vi "2636 EPSC Pulse Sweep.vi"() -> ()   [LabVIEW 2023]
uses:
  <instrlib>/Keithley 2600 Series/Public/Channel.ctl
  <instrlib>/Keithley 2600 Series/Keithley 2600 Series.lvlib
  <userlib>/_OpenG.lib/time/time.llb/openg_time.lvlib
panel:
  in  "Pulse Level Step (V)":dbl=1.0
  in  "error in (no error)":errorcluster
  in  "Log Time After Pulses (s)":dbl=0.5 format="%#_13g"
  in  "Log Time Before Pulses (s)":dbl=0.5 format="%#_13g"
  in  "Auto Enable Output":bool=TRUE
  in  "Reset":bool=TRUE
  in  "Error Query":bool
  out "Pulsed IV Filename Out":path caption="Filename Out"
  in  "Pulsed IV Filename":path=path "C:/Data/pulse_I_V.lvm" caption="Filename"
  out "Pulse IV":cluster{"X":dbl[], "Y":dbl[]}[](graph)
  out "I_ds Log Filename Out":path caption="Filename Out"
  in  "I_ds Log Filename":path=path "C:/Data/I_ds_vs_time.lvm" caption="Filename"
  out "Data":dbl[](array[numeric])
  out "Result Chart":dynamicdata(graph)
  out "error out":errorcluster
  out "Complete?":bool
  out "Overflow?":bool
  in  "Stop":bool
  in  "Pulse Duration (s)":dbl=0.01
  in  "Post-Pulse Duration (s)":dbl=0.05
  in  "Pre-Pulse Duration (s)":dbl=0.05
  in  "Buffer size":u32=1024
  in  "Pulse Number":u32=10
  in  "Drain Source Channel":T1=enum."Channel B"
  in  "V_ds(V)":dbl=0.01
  in  "I_ds NPLC":dbl=0.1
  in  "I_ds Range (A)":dbl=1e-06
  in  "I pulse Range (A)":dbl=1e-06
  in  "I pulse NPLC":dbl=0.1
  in  "Pulse Level Start (V)":dbl=1.0
  in  "Pulse Channel":T1
  in  "2636 Address":refnum<visa-resource-name>="GPIB0::26::INSTR"
  # "Synaptic EPSC Pulse Sweep Measurement (Three-terminal Devices)"
  # "by JHC (20250322)"
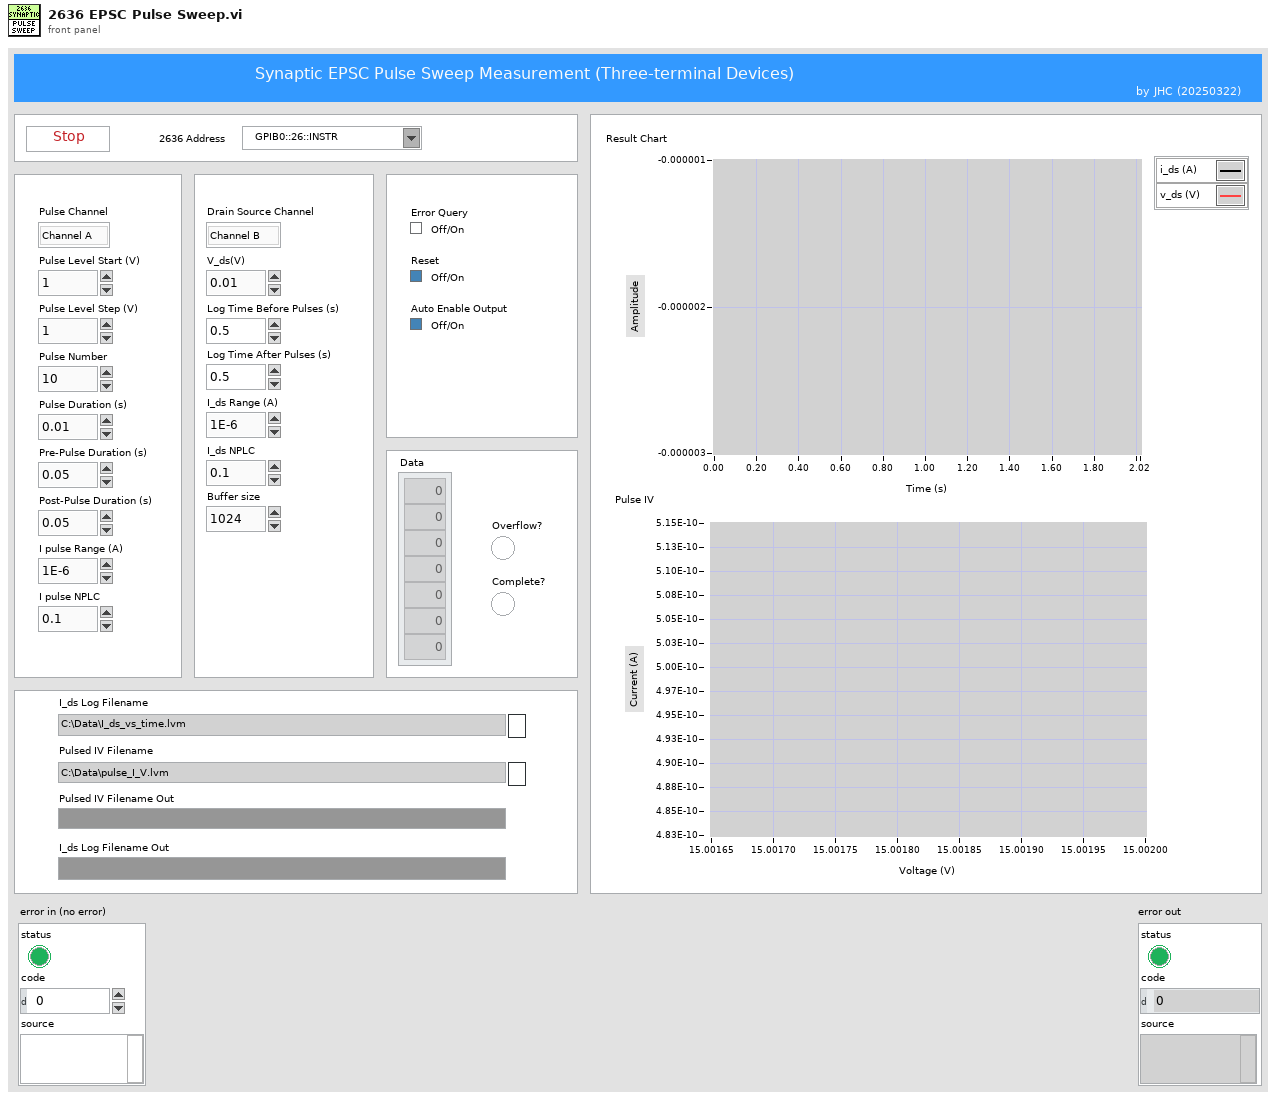
[diagram p1: front panel]
types:
  T1 = typedef "Keithley 2600 Series.lvlib/Channel.ctl" = enum32{"Channel A", "Channel B"}
  T2 = enum16{"None/Disconnect", "Digital I/O Trigger", "TSP-Link Trigger", "LAN Trigger", "Blender", "Timer Expired", "Front Panel Trigger", "Software Trigger", "SMU Sweeping", "SMU Armed", "SMU Source Complete", "SMU Measure Complete", "SMU Pulse Complete", "SMU Sweep Complete", "SMU Idle"}
  T3 = enum16{"Current", "Voltage", "IV", "Resistance", "Power"}
  T4 = enum32{"ASCII", "Real 32", "Real 64", "Single Precision Real", "Double Precision Real"}
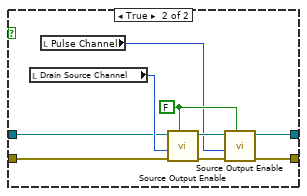
[diagram p2: hidden frame]
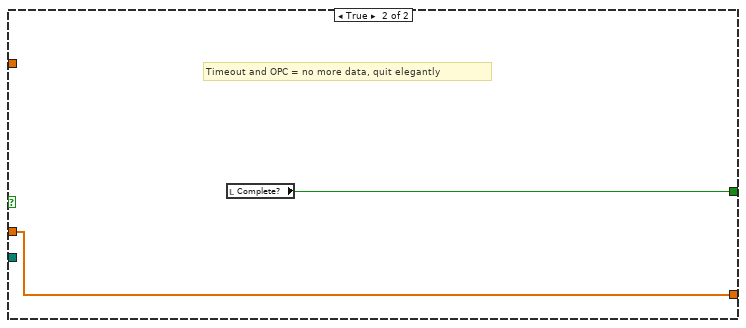
[diagram p5: hidden frame]
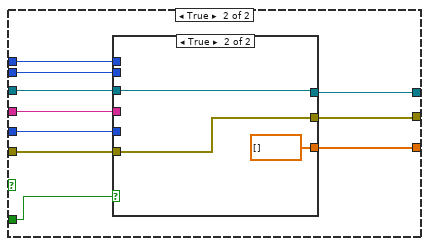
[diagram p8: hidden frame]
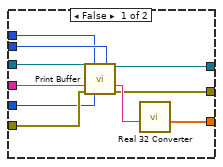
[diagram p9: hidden frame]
diagram:
  w19 = sgl[] [] ("Data Array Out")
  w22 = u16 1 items=["Channel A", "Channel B"] ("Channel (Channel A)")
  w23 = u16 0 items=["Channel A", "Channel B"] ("Channel (Channel A)")
  w39 = u16 0 items=["Current", "Voltage", "Resistance", "Power"] ("Function (Current)")
  w47 = u16 2 items=["Channel A", "Channel B", "Channels A & B", "User"] ("Screen (Channels A & B)")
  # "Wait 1s"
  # "Start Pulse SMU"
  # "Start DS SMU"
  n1 = call <instrlib>:"Initialize.vi"("Reset (True)"="Reset", "error in (no error)"="error in (no error)", "Error Query (False)"="Error Query", "ID Query (True)"=TRUE, "VISA resource name"="2636 Address") -> ("error out"=w2:errorcluster, "VISA resource name out"=w5:refnum<visa-resource-name>)  [unwired: 5 in]
  n2 = call <instrlib>:"Error Queue Clear.vi"("error in (no error)"=w2, "VISA resource name"=w5) -> ("error out"=w3:errorcluster, "VISA resource name out"=w4:refnum<visa-resource-name>)  [unwired: 6 in, 2 out]
  n3 = call <instrlib>:"Abort SMU Op.vi"("error in"=w3, "Channel (Channel A)"=w23, "VISA resource name"=w4) -> ("error out"=w24:errorcluster, "VISA resource name out"=w25:refnum<visa-resource-name>)  [unwired: 5 in, 2 out]
  n4 = call <instrlib>:"Abort SMU Op.vi"("error in"=w24, "Channel (Channel A)"=w22, "VISA resource name"=w25) -> ("error out"=w20:errorcluster, "VISA resource name out"=w21:refnum<visa-resource-name>)  [unwired: 5 in, 2 out]
  n5 = call <instrlib>:"Reset SMU.vi"("SMU B (No)"="Reset", "SMU A (No)"="Reset", "error in (no error)"=w20, "VISA resource name"=w21) -> ("error out"=w86:errorcluster, "VISA resource name out"=w87:refnum<visa-resource-name>)  [unwired: 4 in, 2 out]
  n6 = flat-sequence {
    tunnel: w87 -> [w120]
    tunnel: w86 -> [w119]
    tunnel: [w101] -> w85
    tunnel: [w100] -> w84
    tunnel: w85 -> [w143]
    tunnel: w84 -> [w144]
    tunnel: [w142] -> w83
    tunnel: [w141] -> w82
    tunnel: w83 -> [w185]
    tunnel: w82 -> [w183]
    tunnel: [w164] -> w81
    tunnel: [w163] -> w80
    tunnel: w81 -> [w269]
    tunnel: w80 -> [w268]
    tunnel: [w236] -> w79
    tunnel: [w235] -> w78
    tunnel: [w221] -> w77
    tunnel: w79 -> [w306]
    tunnel: w78 -> [w307]
    tunnel: w77 -> [w329]
    tunnel: [w310] -> w76
    tunnel: [w309] -> w75
    tunnel: w76 -> [w337]
    tunnel: w75 -> [w336]
    tunnel: [w333] -> w44
    tunnel: [w332] -> w43
    frame #0 {
      w108 = enum32{"Current", "Voltage"}."Current" ("Function (Current)")
      w109 = FALSE ("Autorange (On)")
      w89 = enum32{"Current", "Voltage"}."Voltage" ("Function (Current)")
      # "Init Pulse Gate Channel"
      n7 = call <instrlib>:"Source Function.vi"("Function (Current)"=w89, "error in (no error)"=w119, "Channel (Channel A)"="Pulse Channel", "VISA resource name"=w120) -> ("error out"=w121:errorcluster, "VISA resource name out"=w122:refnum<visa-resource-name>)  [unwired: 4 in, 2 out]
      n8 = call <instrlib>:"Source Level.vi"("Level (0.000)"=0.0, "Function (Current)"=w89, "error in (no error)"=w121, "Channel (Channel A)"="Pulse Channel", "VISA resource name"=w122) -> ("error out"=w117:errorcluster, "VISA resource name out"=w118:refnum<visa-resource-name>)  [unwired: 3 in, 2 out]
      n9 = call <instrlib>:"Source Autorange.vi"("Autorange (On)"=w109, "Function (Current)"=w89, "error in (no error)"=w117, "Channel (Channel A)"="Pulse Channel", "VISA resource name"=w118) -> ("error out"=w115:errorcluster, "VISA resource name out"=w116:refnum<visa-resource-name>)  [unwired: 3 in, 2 out]
      n10 = local read "Pulse Level Start (V)"() -> (w88:dbl)
      n11 = call <instrlib>:"Source Autorange.vi"("Autorange (On)"=w109, "Function (Current)"=w108, "error in (no error)"=w115, "Channel (Channel A)"="Pulse Channel", "VISA resource name"=w116) -> ("error out"=w96:errorcluster, "VISA resource name out"=w98:refnum<visa-resource-name>)  [unwired: 3 in, 2 out]
      n12 = call <instrlib>:"Source Range.vi"("Range (1.000)"=w88, "Function (Current)"=w89, "error in (no error)"=w96, "Channel (Channel A)"="Pulse Channel", "VISA resource name"=w98) -> ("error out"=w95:errorcluster, "VISA resource name out"=w97:refnum<visa-resource-name>)  [unwired: 3 in, 2 out]
      n13 = call <instrlib>:"Measure NPLC.vi"("NPLC (1.000)"="I pulse NPLC", "error in (no error)"=w95, "Channel (Channel A)"="Pulse Channel", "VISA resource name"=w97) -> ("error out"=w113:errorcluster, "VISA resource name out"=w110:refnum<visa-resource-name>)  [unwired: 4 in, 2 out]
      n14 = call <instrlib>:"Measure Autorange.vi"("Autorange (On)"=w109, "Function (Current)"=w89, "error in (no error)"=w113, "Channel (Channel A)"="Pulse Channel", "VISA resource name"=w110) -> ("error out"=w112:errorcluster, "VISA resource name out"=w111:refnum<visa-resource-name>)  [unwired: 3 in, 2 out]
      n15 = call <instrlib>:"Measure Autorange.vi"("Autorange (On)"=w109, "Function (Current)"=w108, "error in (no error)"=w112, "Channel (Channel A)"="Pulse Channel", "VISA resource name"=w111) -> ("error out"=w94:errorcluster, "VISA resource name out"=w93:refnum<visa-resource-name>)  [unwired: 3 in, 2 out]
      n16 = call <instrlib>:"Measure Range.vi"("Range (1.000)"=w88, "Function (Current)"=w89, "error in (no error)"=w94, "Channel (Channel A)"="Pulse Channel", "VISA resource name"=w93) -> ("error out"=w91:errorcluster, "VISA resource name out"=w92:refnum<visa-resource-name>)  [unwired: 3 in, 2 out]
      n17 = call <instrlib>:"Measure Range.vi"("Range (1.000)"="I pulse Range (A)", "Function (Current)"=w108, "error in (no error)"=w91, "Channel (Channel A)"="Pulse Channel", "VISA resource name"=w92) -> ("error out"=w106:errorcluster, "VISA resource name out"=w105:refnum<visa-resource-name>)  [unwired: 3 in, 2 out]
      n18 = call <instrlib>:"Measure Sense Mode.vi"("error in (no error)"=w106, "Channel (Channel A)"="Pulse Channel", "VISA resource name"=w105) -> ("error out"=w103:errorcluster, "VISA resource name out"=w104:refnum<visa-resource-name>)  [unwired: 2 in, 5 out]
      n19 = call <instrlib>:"Measure Autozero.vi"("Autozero (Auto)"=enum32{"Off", "Once", "Auto"}."Once", "error in (no error)"=w103, "Channel (Channel A)"="Pulse Channel", "VISA resource name"=w104) -> ("error out"=w100:errorcluster, "VISA resource name out"=w101:refnum<visa-resource-name>)  [unwired: 1 in, 5 out]
    }
    frame #1 {
      w126 = 0.0 ("Interval (0.000)")
      w146 = enum32{"Current", "Voltage"}."Current" ("Function (Current)")
      w145 = FALSE ("Autorange (On)")
      w132 = enum32{"Current", "Voltage"}."Voltage" ("Function (Current)")
      # "Init Drain Source Channel"
      n20 = call <instrlib>:"Source Function.vi"("Function (Current)"=w132, "error in (no error)"=w144, "Channel (Channel A)"="Drain Source Channel", "VISA resource name"=w143) -> ("error out"=w160:errorcluster, "VISA resource name out"=w161:refnum<visa-resource-name>)  [unwired: 4 in, 2 out]
      n21 = call <instrlib>:"Source Level.vi"("Level (0.000)"="V_ds(V)", "Function (Current)"=w132, "error in (no error)"=w160, "Channel (Channel A)"="Drain Source Channel", "VISA resource name"=w161) -> ("error out"=w158:errorcluster, "VISA resource name out"=w159:refnum<visa-resource-name>)  [unwired: 3 in, 2 out]
      n22 = call <instrlib>:"Source Autorange.vi"("Autorange (On)"=w145, "Function (Current)"=w132, "error in (no error)"=w158, "Channel (Channel A)"="Drain Source Channel", "VISA resource name"=w159) -> ("error out"=w156:errorcluster, "VISA resource name out"=w157:refnum<visa-resource-name>)  [unwired: 3 in, 2 out]
      n23 = call <instrlib>:"Source Autorange.vi"("Autorange (On)"=w145, "Function (Current)"=w146, "error in (no error)"=w156, "Channel (Channel A)"="Drain Source Channel", "VISA resource name"=w157) -> ("error out"=w140:errorcluster, "VISA resource name out"=w137:refnum<visa-resource-name>)  [unwired: 3 in, 2 out]
      n24 = call <instrlib>:"Source Range.vi"("Range (1.000)"="V_ds(V)", "Function (Current)"=w132, "error in (no error)"=w140, "Channel (Channel A)"="Drain Source Channel", "VISA resource name"=w137) -> ("error out"=w139:errorcluster, "VISA resource name out"=w138:refnum<visa-resource-name>)  [unwired: 3 in, 2 out]
      n25 = call <instrlib>:"Measure NPLC.vi"("NPLC (1.000)"="I_ds NPLC", "error in (no error)"=w139, "Channel (Channel A)"="Drain Source Channel", "VISA resource name"=w138) -> ("error out"=w127:errorcluster, "VISA resource name out"=w128:refnum<visa-resource-name>)  [unwired: 4 in, 2 out]
      n26 = call <instrlib>:"Measure Interval.vi"("Interval (0.000)"=w126, "error in (no error)"=w127, "Channel (Channel A)"="Drain Source Channel", "VISA resource name"=w128) -> ("error out"=w130:errorcluster, "VISA resource name out"=w129:refnum<visa-resource-name>)  [unwired: 4 in, 2 out]
      n27 = call <instrlib>:"Measure Delay.vi"("Delay (0)"=w126, "error in (no error)"=w130, "Channel (Channel A)"="Drain Source Channel", "VISA resource name"=w129) -> ("error out"=w124:errorcluster, "VISA resource name out"=w125:refnum<visa-resource-name>)  [unwired: 4 in, 2 out]
      n28 = call <instrlib>:"Measure Autorange.vi"("Autorange (On)"=w145, "Function (Current)"=w132, "error in (no error)"=w124, "Channel (Channel A)"="Drain Source Channel", "VISA resource name"=w125) -> ("error out"=w154:errorcluster, "VISA resource name out"=w153:refnum<visa-resource-name>)  [unwired: 3 in, 2 out]
      n29 = call <instrlib>:"Measure Autorange.vi"("Autorange (On)"=w145, "Function (Current)"=w146, "error in (no error)"=w154, "Channel (Channel A)"="Drain Source Channel", "VISA resource name"=w153) -> ("error out"=w133:errorcluster, "VISA resource name out"=w134:refnum<visa-resource-name>)  [unwired: 3 in, 2 out]
      n30 = call <instrlib>:"Measure Range.vi"("Range (1.000)"="V_ds(V)", "Function (Current)"=w132, "error in (no error)"=w133, "Channel (Channel A)"="Drain Source Channel", "VISA resource name"=w134) -> ("error out"=w136:errorcluster, "VISA resource name out"=w135:refnum<visa-resource-name>)  [unwired: 3 in, 2 out]
      n31 = call <instrlib>:"Measure Range.vi"("Range (1.000)"="I_ds Range (A)", "Function (Current)"=w146, "error in (no error)"=w136, "VISA resource name"=w135) -> ("error out"=w151:errorcluster, "VISA resource name out"=w150:refnum<visa-resource-name>)  [unwired: 4 in, 2 out]
      n32 = call <instrlib>:"Measure Sense Mode.vi"("error in (no error)"=w151, "Channel (Channel A)"="Drain Source Channel", "VISA resource name"=w150) -> ("error out"=w148:errorcluster, "VISA resource name out"=w149:refnum<visa-resource-name>)  [unwired: 2 in, 5 out]
      n33 = call <instrlib>:"Measure Autozero.vi"("Autozero (Auto)"=enum32{"Off", "Once", "Auto"}."Once", "error in (no error)"=w148, "Channel (Channel A)"="Drain Source Channel", "VISA resource name"=w149) -> ("error out"=w142:errorcluster, "VISA resource name out"=w141:refnum<visa-resource-name>)  [unwired: 1 in, 5 out]
    }
    frame #2 {
      w177 = TRUE ("Append Mode (Off)")
      w176 = "v_ds" ("Buffer Name (buf)")
      w178 = TRUE ("Append Mode (Off)")
      w180 = "i_ds" ("Buffer Name (buf)")
      w189 = FALSE ("Collect Timestamps (Off)")
      w188 = "pulse_iv_table.v" ("Buffer Name (buf)")
      w187 = TRUE ("Append Mode (Off)")
      w186 = "pulse_iv_table.i" ("Buffer Name (buf)")
      # "set up circular buffer"
      # "A large size"
      # "Init Buffer"
      n34 = local read "Pulse Channel"() -> (w204:T1)
      n35 = VISA Write(VISA resource name=w183, write buffer="pulse_iv_table = {}\nds_iv_table = {}", error in (no error)=w185) -> (VISA resource name out=w190:refnum<visa-resource-name>, error out=w191:errorcluster)  [unwired: 1 out]
      n36 = local read "Pulse Number"() -> (w162:u32)
      n37 = call <instrlib>:"Error Query.vi"("error in (no error)"=w191, "VISA resource name"=w190) -> ("error out"=w203:errorcluster, "VISA resource name out"=w202:refnum<visa-resource-name>)  [unwired: 8 out]
      n38 = call <instrlib>:"Buffer Make Buffer.vi"("Capacity (1)"=w162, "Channel (Channel A)"=w204, "error in (no error)"=w203, "Buffer Name (buf)"=w186, "VISA resource name"=w202) -> ("error out"=w192:errorcluster, "VISA resource name out"=w193:refnum<visa-resource-name>)  [unwired: 1 in, 4 out]
      n39 = call <instrlib>:"Buffer Clear.vi"("error in (no error)"=w192, "Buffer Name"=w186, "VISA resource name"=w193) -> ("error out"=w195:errorcluster, "VISA resource name out"=w194:refnum<visa-resource-name>)  [unwired: 7 out]
      n40 = call <instrlib>:"Buffer Configure.vi"("Collect Timestamps (Off)"=w189, "error in (no error)"=w195, "Buffer Name"=w186, "Append Mode (Off)"=w187, "VISA resource name"=w194) -> ("error out"=w197:errorcluster, "VISA resource name out"=w196:refnum<visa-resource-name>)  [unwired: 2 in, 3 out]
      n41 = call <instrlib>:"Buffer Make Buffer.vi"("Capacity (1)"=w162, "Channel (Channel A)"=w204, "error in (no error)"=w197, "Buffer Name (buf)"=w188, "VISA resource name"=w196) -> ("error out"=w199:errorcluster, "VISA resource name out"=w198:refnum<visa-resource-name>)  [unwired: 1 in, 4 out]
      n42 = call <instrlib>:"Buffer Clear.vi"("error in (no error)"=w199, "Buffer Name"=w188, "VISA resource name"=w198) -> ("error out"=w201:errorcluster, "VISA resource name out"=w200:refnum<visa-resource-name>)  [unwired: 7 out]
      n43 = call <instrlib>:"Buffer Configure.vi"("Collect Source Values (Off)"=w189, "error in (no error)"=w201, "Buffer Name"=w188, "Append Mode (Off)"=w187, "VISA resource name"=w200) -> ("error out"=w210:errorcluster, "VISA resource name out"=w209:refnum<visa-resource-name>)  [unwired: 2 in, 3 out]
      n44 = local read "Drain Source Channel"() -> (w168:T1)
      n45 = call <instrlib>:"Buffer Make Buffer.vi"("Capacity (1)"="Buffer size", "Channel (Channel A)"=w168, "error in (no error)"=w210, "Buffer Name (buf)"=w180, "VISA resource name"=w209) -> ("error out"=w206:errorcluster, "VISA resource name out"=w205:refnum<visa-resource-name>)  [unwired: 1 in, 4 out]
      n46 = call <instrlib>:"Buffer Clear.vi"("error in (no error)"=w206, "Buffer Name"=w180, "VISA resource name"=w205) -> ("error out"=w208:errorcluster, "VISA resource name out"=w207:refnum<visa-resource-name>)  [unwired: 7 out]
      n47 = call <instrlib>:"Buffer Configure.vi"("Collect Timestamps (Off)"=w178, "error in (no error)"=w208, "Buffer Name"=w180, "Append Mode (Off)"=w178, "VISA resource name"=w207) -> ("error out"=w182:errorcluster, "VISA resource name out"=w181:refnum<visa-resource-name>)  [unwired: 2 in, 3 out]
      n48 = call <instrlib>:"Advanced Buffer Configuration.vi"("VISA resource name"=w181, "Enable Buffer Cache Mode (Disable)"=w178, "Buffer Name"=w180, "Buffer Fill Mode (Fill_Once)"=enum16{"FILL_ONCE", "FILL_WINDOW"}."FILL_WINDOW", "error in (no error)"=w182) -> ("VISA resource name out"=w166:refnum<visa-resource-name>, "error out"=w165:errorcluster)  [unwired: 9 in]
      n49 = call <instrlib>:"Buffer Make Buffer.vi"("Capacity (1)"="Buffer size", "Channel (Channel A)"=w168, "error in (no error)"=w165, "Buffer Name (buf)"=w176, "VISA resource name"=w166) -> ("error out"=w172:errorcluster, "VISA resource name out"=w173:refnum<visa-resource-name>)  [unwired: 1 in, 4 out]
      n50 = call <instrlib>:"Buffer Clear.vi"("error in (no error)"=w172, "Buffer Name"=w176, "VISA resource name"=w173) -> ("error out"=w170:errorcluster, "VISA resource name out"=w171:refnum<visa-resource-name>)  [unwired: 7 out]
      n51 = call <instrlib>:"Buffer Configure.vi"("Collect Timestamps (Off)"=w177, "error in (no error)"=w170, "Buffer Name"=w176, "Append Mode (Off)"=w177, "VISA resource name"=w171) -> ("error out"=w174:errorcluster, "VISA resource name out"=w175:refnum<visa-resource-name>)  [unwired: 2 in, 3 out]
      n52 = call <instrlib>:"Advanced Buffer Configuration.vi"("VISA resource name"=w175, "Enable Buffer Cache Mode (Disable)"=w177, "Buffer Name"=w176, "Buffer Fill Mode (Fill_Once)"=enum16{"FILL_ONCE", "FILL_WINDOW"}."FILL_WINDOW", "error in (no error)"=w174) -> ("VISA resource name out"=w163:refnum<visa-resource-name>, "error out"=w164:errorcluster)  [unwired: 9 in]
    }
    frame #3 {
      w225 = u32 4 ("Timer Number (1)")
      w239 = u32 1 ("Timer Number (1)")
      w251 = u32 3 ("Timer Number (1)")
      w274 = u32 2 ("Timer Number (1)")
      # "SMU Armed when timer4 expires"
      # "Trigger timer4 when the SMU Sweeping, only once"
      # "Trigger timer1 when the SMU Armed, repeat N times"
      # "Trigger end pulse after timer3 expired"
      # "Configure measure action (default is 0) to start after source immediately"
      # "set source pulse level and end pusle idle"
      # "Trigger timer3 when the SMU source pulse level"
      # "Create a fixed level voltage sweep"
      # "Configure source action to start after timer2 expired"
      # "Trigger timer2 when timer1 expired or first run."
      # "Init Trigger Model (Pulse Channel)"
      n53 = for {
        N: "Pulse Number" -> [_]
        tunnel: "Pulse Level Start (V)" -> [w284]
        tunnel: "Pulse Level Step (V)" -> [w285]
        tunnel: [w282] -> w212 mode=indexing
        i -> [w286]
        n54 = Multiply(x=w285, y=w286) -> (x*y=w283:dbl)
        n55 = Add(x=w284, y=w283) -> (x+y=w282:dbl)
      }
      n56 = Array To Spreadsheet String(delimiter (Tab)=",", array=w212, 3:"%f" ("format string")) -> (spreadsheet string=w211:string)
      n57 = local read "Pulse Channel"() -> (w221:T1)
      n58 = Pick Line(multi-line string="smua\nsmub", line index=w221) -> (output string=w234:string)  [unwired: 1 in]
      n59 = Format Into String(format string="%s.trigger.source.listv({%s})\\n", w234, w211) -> (resulting string=w272:string)  [unwired: 2 in, 1 out]
      n60 = call <instrlib>:"Format Event ID.vi"("Channel (Channel A)"=w221, "Event Type (None)"=T2."SMU Sweeping") -> ("Event ID"=w229:string)  [unwired: 8 in, 1 out]
      n61 = Format Into String(format string="%s.trigger.source.action = %s.ENABLE\n%s.trigger.endpulse.action = %s.SOURCE_IDLE", initial string=w272, w234, w234, w234, w234) -> (resulting string=w267:string)  [unwired: 1 in, 1 out]
      n62 = VISA Write(VISA resource name=w268, write buffer=w267, error in (no error)=w269) -> (VISA resource name out=w231:refnum<visa-resource-name>, error out=w230:errorcluster)  [unwired: 1 out]
      n63 = call <instrlib>:"Config Timer.vi"("VISA resource name"=w231, "Delay (1e-3)"="Log Time Before Pulses (s)", "Timer Number (1)"=w225, "error in"=w230, "Input Event"=w229) -> ("VISA resource name out"=w227:refnum<visa-resource-name>, "error out"=w223:errorcluster)  [unwired: 7 in, 2 out]
      n64 = call <instrlib>:"Format Event ID.vi"("Event Module # (1)"=w225, "Event Type (None)"=T2."Timer Expired") -> ("Event ID"=w224:string)  [unwired: 8 in, 1 out]
      n65 = call <instrlib>:"Config Arm Event.vi"("Arm Input Event"=w224, "error in"=w223, "Channel (Channel A)"=w221, "VISA resource name"=w227) -> ("error out"=w219:errorcluster, "VISA resource name out"=w218:refnum<visa-resource-name>)  [unwired: 4 in, 2 out]
      n66 = call <instrlib>:"Format Event ID.vi"("Channel (Channel A)"=w221, "Event Type (None)"=T2."SMU Armed") -> ("Event ID"=w220:string)  [unwired: 8 in, 1 out]
      n67 = local read "Pre-Pulse Duration (s)"() -> (w248:dbl)
      n68 = local read "Pulse Number"() -> (w244:u32)
      n69 = local read "Pulse Duration (s)"() -> (w249:dbl)
      n70 = Decrement(x=w244) -> (x-1=w240:u32)
      n71 = Compound Arithmetic op=ADD(w249, w248, "Post-Pulse Duration (s)") -> (w246:dbl)
      n72 = call <instrlib>:"Config Timer.vi"("VISA resource name"=w218, "Count (1)"=w240, "Delay (1e-3)"=w246, "Timer Number (1)"=w239, "Passthrough (Off)"=TRUE, "error in"=w219, "Input Event"=w220) -> ("VISA resource name out"=w241:refnum<visa-resource-name>, "error out"=w242:errorcluster)  [unwired: 5 in, 2 out]
      n73 = call <instrlib>:"Format Event ID.vi"("Event Module # (1)"=w239, "Event Type (None)"=T2."Timer Expired") -> ("Event ID"=w278:string)  [unwired: 8 in, 1 out]
      n74 = call <instrlib>:"Config Timer.vi"("VISA resource name"=w241, "Delay (1e-3)"="Pre-Pulse Duration (s)", "Timer Number (1)"=w274, "error in"=w242, "Input Event"=w278) -> ("VISA resource name out"=w277:refnum<visa-resource-name>, "error out"=w276:errorcluster)  [unwired: 7 in, 2 out]
      n75 = call <instrlib>:"Format Event ID.vi"("Event Module # (1)"=w274, "Event Type (None)"=T2."Timer Expired") -> ("Event ID"=w273:string)  [unwired: 8 in, 1 out]
      n76 = call <instrlib>:"Config Source Event.vi"("Input Event"=w273, "error in"=w276, "Channel (Channel A)"=w221, "VISA resource name"=w277) -> ("error out"=w262:errorcluster, "VISA resource name out"=w263:refnum<visa-resource-name>)  [unwired: 4 in, 2 out]
      n77 = call <instrlib>:"Format Event ID.vi"("Channel (Channel A)"=w221, "Event Type (None)"=T2."SMU Source Complete") -> ("Event ID"=w265:string)  [unwired: 8 in, 1 out]
      n78 = call <instrlib>:"Config Timer.vi"("VISA resource name"=w263, "Delay (1e-3)"="Pulse Duration (s)", "Timer Number (1)"=w251, "error in"=w262, "Input Event"=w265) -> ("VISA resource name out"=w261:refnum<visa-resource-name>, "error out"=w260:errorcluster)  [unwired: 7 in, 2 out]
      n79 = call <instrlib>:"Config Measure Event.vi"("VISA resource name"=w261, "Configure Measurement (Disable)"=enum8{"DISABLE", "ENABLE", "ASYNC"}."ENABLE", "Buffer 1"="pulse_iv_table.i" ("Buffer Name (buf)"), "Buffer 2"="pulse_iv_table.v" ("Buffer Name (buf)"), "Channel (Channel A)"=w221, "Function (Current)"=T3."IV", "error in"=w260, "Measure Input Event"="0") -> ("VISA resource name out"=w254:refnum<visa-resource-name>, "error out"=w253:errorcluster)  [unwired: 4 in, 2 out]
      n80 = call <instrlib>:"Format Event ID.vi"("Event Module # (1)"=w251, "Event Type (None)"=T2."Timer Expired") -> ("Event ID"=w250:string)  [unwired: 8 in, 1 out]
      n81 = local read "Pulse Number"() -> (w232:u32)
      n82 = call <instrlib>:"Config End Pulse Event.vi"("Input Event"=w250, "error in"=w253, "Channel (Channel A)"=w221, "VISA resource name"=w254) -> ("error out"=w238:errorcluster, "VISA resource name out"=w237:refnum<visa-resource-name>)  [unwired: 4 in, 2 out]
      n83 = call <instrlib>:"Config Layer Count.vi"("Trigger Count (1)"=w232, "Arm Count (1)"=u32 1 ("Trigger Count (1)"), "error in"=w238, "Channel (Channel A)"=w221, "VISA resource name"=w237) -> ("error out"=w235:errorcluster, "VISA resource name out"=w236:refnum<visa-resource-name>)  [unwired: 3 in, 2 out]
    }
    frame #4 {
      w291 = u32 5 ("Timer Number (1)")
      w319 = u32 1 ("Blender Number (1)")
      # "BUG from Driver: if Async, measure.Y is not set"
      # "No trigger, start\nasync measure after SMU Armed, as fast as possible"
      # "Trigger timer5 when Pulse SMU Idle\nto keep measure for a while"
      # "Blend two events from Pulse SMU to trigger DS SMU Source action\nDS SMU Source start when Pulse SMU start sweeping\nWhen Pulse SMU become idle, DS SMU source again and stop"
      # "set source level, and hold"
      # "Create a fixed level voltage sweep"
      # "Init Trigger Model (Drain Source Channel)"
      n84 = local read "Drain Source Channel"() -> (w312:T1)
      n85 = local read "V_ds(V)"() -> (w323:dbl)
      n86 = Pick Line(multi-line string="smua\nsmub", line index=w312) -> (output string=w299:string)  [unwired: 1 in]
      n87 = Format Into String(format string="%s.trigger.source.listv({%f})\\n", w299, w323) -> (resulting string=w326:string)  [unwired: 2 in, 1 out]
      n88 = Format Into String(format string="%s.trigger.source.action = %s.ENABLE\n%s.trigger.endpulse.action = %s.SOURCE_HOLD", initial string=w326, w299, w299, w299, w299) -> (resulting string=w305:string)  [unwired: 1 in, 1 out]
      n89 = VISA Write(VISA resource name=w306, write buffer=w305, error in (no error)=w307) -> (VISA resource name out=w295:refnum<visa-resource-name>, error out=w296:errorcluster)  [unwired: 1 out]
      n90 = call <instrlib>:"Format Event ID.vi"("Channel (Channel A)"=w329, "Event Type (None)"=T2."SMU Sweeping") -> ("Event ID"=w290:string)  [unwired: 8 in, 1 out]
      n91 = call <instrlib>:"Format Event ID.vi"("Channel (Channel A)"=w329, "Event Type (None)"=T2."SMU Idle") -> ("Event ID"=w293:string)  [unwired: 8 in, 1 out]
      n92 = call <instrlib>:"Config Timer.vi"("VISA resource name"=w295, "Delay (1e-3)"="Log Time After Pulses (s)", "Timer Number (1)"=w291, "error in"=w296, "Input Event"=w293) -> ("VISA resource name out"=w287:refnum<visa-resource-name>, "error out"=w288:errorcluster)  [unwired: 7 in, 2 out]
      n93 = call <instrlib>:"Format Event ID.vi"("Event Module # (1)"=w291, "Event Type (None)"=T2."Timer Expired") -> ("Event ID"=w289:string)  [unwired: 8 in, 1 out]
      n94 = call <instrlib>:"Config Event Blender.vi"("VISA resource name"=w287, "Input Event 1"=w289, "Input Event 2"=w290, "Blender Number (1)"=w319, "Blend Type (OR)"=enum16{"OR", "AND"}."OR", "error in"=w288) -> ("VISA resource name out"=w321:refnum<visa-resource-name>, "error out"=w322:errorcluster)  [unwired: 6 in, 2 out]
      n95 = call <instrlib>:"Format Event ID.vi"("Event Module # (1)"=w319, "Event Type (None)"=T2."Blender") -> ("Event ID"=w318:string)  [unwired: 8 in, 1 out]
      n96 = call <instrlib>:"Config Source Event.vi"("Input Event"=w318, "error in"=w322, "Channel (Channel A)"=w312, "VISA resource name"=w321) -> ("error out"=w315:errorcluster, "VISA resource name out"=w316:refnum<visa-resource-name>)  [unwired: 4 in, 2 out]
      n97 = call <instrlib>:"Config Measure Event.vi"("VISA resource name"=w316, "Configure Measurement (Disable)"=enum8{"DISABLE", "ENABLE", "ASYNC"}."ENABLE", "Buffer 1"="i_ds" ("Buffer Name (buf)"), "Buffer 2"="v_ds" ("Buffer Name (buf)"), "Channel (Channel A)"=w312, "Function (Current)"=T3."IV", "error in"=w315) -> ("VISA resource name out"=w301:refnum<visa-resource-name>, "error out"=w302:errorcluster)  [unwired: 5 in, 2 out]
      n98 = Format Into String(format string="%s.trigger.measure.action = %s.ASYNC", w299, w299) -> (resulting string=w298:string)  [unwired: 2 in, 1 out]
      n99 = VISA Write(VISA resource name=w301, write buffer=w298, error in (no error)=w302) -> (VISA resource name out=w304:refnum<visa-resource-name>, error out=w303:errorcluster)  [unwired: 1 out]
      n100 = call <instrlib>:"Config Layer Count.vi"("Trigger Count (1)"=u32 2 ("Arm Count (1)"), "Arm Count (1)"=u32 1, "error in"=w303, "Channel (Channel A)"=w312, "VISA resource name"=w304) -> ("error out"=w309:errorcluster, "VISA resource name out"=w310:refnum<visa-resource-name>)  [unwired: 3 in, 2 out]
    }
    frame #5 {
      # "Other init jobs"
      n101 = call <instrlib>:"Data Output Format.vi"("ASCII Precision (6)"=6, "error in (no error)"=w336, "Data Format (ASCII)"=T4."Real 32", "VISA resource name"=w337) -> ("error out"=w332:errorcluster, "VISA resource name out"=w333:refnum<visa-resource-name>)  [unwired: 4 in, 2 out]
    }
  }
  n102 = local read "Pulse Channel"() -> (w41:T1)
  n103 = local read "Drain Source Channel"() -> (w40:T1)
  n104 = call <instrlib>:"Display Screen.vi"("Screen (Channels A & B)"=w47, "error in (no error)"=w43, "VISA resource name"=w44) -> ("error out"=w50:errorcluster, "Node Out"=w49:string, "VISA resource name out"=w48:refnum<visa-resource-name>)  [unwired: 5 in, 1 out]
  n105 = call <instrlib>:"Display Measure Function.vi"("Function (Current)"=w39, "error in (no error)"=w50, "Channel (Channel A)"=w41, "Node In"=w49, "VISA resource name"=w48) -> ("error out"=w46:errorcluster, "VISA resource name out"=w45:refnum<visa-resource-name>)  [unwired: 3 in, 2 out]
  n106 = control-ref of="Overflow?"() -> (w36:refnum<vi>)
  n107 = control-ref of="Complete?"() -> (w35:refnum<vi>)
  n108 = control-ref of="Stop"() -> (w30:refnum<vi>)
  n109 = call <instrlib>:"Display Measure Function.vi"("Function (Current)"=w39, "error in (no error)"=w46, "Channel (Channel A)"=w40, "VISA resource name"=w45) -> ("error out"=w42:errorcluster, "VISA resource name out"=w38:refnum<visa-resource-name>)  [unwired: 4 in, 2 out]
  n110 = Build Array(w36, w35, w30) -> (w34:refnum<vi>[])
  n111 = case shown="True" "Auto Enable Output" {
    tunnel: [w338 w348] -> w9
    tunnel: [w339 w347] -> w10
    tunnel: w42 -> [w338 w343]
    tunnel: w41 -> [_ w342]
    tunnel: w40 -> [_ w341]
    tunnel: w38 -> [w339 w340]
    frame False {
    }
    frame True {
      w344 = TRUE ("Output (Off)")
      n112 = call <instrlib>:"Source Output Enable.vi"("Output (Off)"=w344, "error in (no error)"=w343, "Channel (Channel A)"=w341, "VISA resource name"=w340) -> ("error out"=w346:errorcluster, "VISA resource name out"=w345:refnum<visa-resource-name>)  [unwired: 4 in, 2 out]
      n113 = call <instrlib>:"Source Output Enable.vi"("Output (Off)"=w344, "error in (no error)"=w346, "Channel (Channel A)"=w342, "VISA resource name"=w345) -> ("error out"=w348:errorcluster, "VISA resource name out"=w347:refnum<visa-resource-name>)  [unwired: 4 in, 2 out]
    }
  }
  n114 = for {
    tunnel: w34 -> [w350] mode=indexing
    tunnel: [w349] -> w31
    # "Init GUI"
    n115 = invoke class="Bool (strict)" method="Reinit To Default"(reference=w350) -> (error out=w349:errorcluster)  [unwired: 2 in, 2 out]
  }
  n116 = call <userlib>:"Wait (ms)__ogtk.vi"("error in (no error)"=w9, "milliseconds to wait"=u32 1000) -> ("error out"=w8:errorcluster)  [unwired: 8 in, 1 out]
  n117 = call <instrlib>:"Initiate Sweep.vi"("error in"=w8, "Channel (Channel A)"=w40, "VISA resource name"=w10) -> ("error out"=w70:errorcluster, "VISA resource name out"=w71:refnum<visa-resource-name>)  [unwired: 5 in, 2 out]
  n118 = Obtain Queue(max queue size (-1, unlimited)=1024, name (unnamed)="data_q", element data type=w19, error in (no error)=w42) -> (queue out=w57:refnum<queue>, error out=w32:errorcluster)  [unwired: 1 in, 1 out]
  n119 = Format Into String(format string="%s, %s, %s", "i_ds" ("Buffer Name(s)"), "i_ds.timestamps" ("Buffer Name(s)"), "v_ds" ("Buffer Name(s)")) -> (resulting string=w74:string)  [unwired: 2 in, 1 out]
  n120 = call <instrlib>:"Initiate Sweep.vi"("error in"=w70, "Channel (Channel A)"=w41, "VISA resource name"=w71) -> ("error out"=w73:errorcluster, "VISA resource name out"=w72:refnum<visa-resource-name>)  [unwired: 5 in, 2 out]
  n121 = Merge Errors(w32, w31) -> (w33:errorcluster)
  n122 = while {
    tunnel: w57 -> [w362]
    tunnel: "I_ds Log Filename" -> [w358]
    tunnel: w33 -> [w361]
    tunnel: [w357] -> w29
    shift-right: [w351] -> w15
    shift-left: w19 -> [w352]
    stop <- w355 stop-if-true
    # "Plot and save I_ds and v_ds"
    n123 = Dequeue Element(queue=w362, timeout in ms (-1)=500, error in (no error)=w361) -> (queue out=w357:refnum<queue>, element=w359:sgl[], timed out?=w360:bool, error out=w354:errorcluster)
    n124 = case shown="False" w360 {
      tunnel: w359 -> [w365 _]
      tunnel: w358 -> [w374 _]
      tunnel: [FALSE ("Operation Complete") w387] -> w353
      tunnel: w352 -> [w366 w386]
      tunnel: [w364 w386] -> w351
      frame False {
        n125 = Decimate 1D Array(w365) -> (w371:sgl[], w370:sgl[], w369:sgl[])
        n126 = for {
          tunnel: [w383] -> w373
          tunnel: [w378] -> w368 mode=indexing
          tunnel: w371 -> [w377] mode=indexing
          tunnel: w370 -> [w376] mode=indexing
          tunnel: w369 -> [w381] mode=indexing
          n127 = To Time Stamp(1:w376) -> (0:w382:timestamp)
          n128 = Build Array(w377) -> (w380:sgl[])
          n129 = Build Array(w381) -> (w379:sgl[])
          n130 = Build Array(w376, w377, w381) -> (w378:sgl[])
          "Data" <- w378
          n131 = Bundle By Name("Y"=w380, "t0"=w382) -> (w385:waveform(sgl))  [unwired: 1 in]
          n132 = Bundle By Name("Y"=w379, "t0"=w382) -> (w384:waveform(sgl))  [unwired: 1 in]
          n133 = Merge Signals(w385, w384) -> (w383:dynamicdata)
        }
        "Result Chart" <- w373
        n134 = Build Array (concatenate)(w366, w365) -> (w364:sgl[])
        n135 = call "Convert to Dynamic Data3"("2D Array"=w368) -> ("Dynamic Data Type"=w372:dynamicdata)  [unwired: 3 in]
        n136 = call "Write To Measurement File"("Signals"=w372, "Filename"=w374) -> ("Filename Out"=→"I_ds Log Filename Out":path)  [unwired: 15 in, 2 out]
      }
      frame True {
        # "Timeout and OPC = no more data, quit elegantly"
        n137 = local read "Complete?"() -> (w387:bool)
      }
    }
    n138 = local read "Stop"() -> (w356:bool)
    n139 = Compound Arithmetic op=OR(w353, w356, w354) -> (w355:bool)
  }
  n140 = while {
    tunnel: w72 -> [w396]
    tunnel: w73 -> [w395]
    shift-right: [w390] -> _
    shift-left: u32 1 ("Start Index (1)") -> [w389]
    tunnel: w74 -> [w412]
    tunnel: "tostring(i_ds.next), tostring(v_ds.next)" ("format string") -> [w410]
    tunnel: w57 -> [w394]
    tunnel: [w409] -> w61
    tunnel: [w393] -> w60
    tunnel: [w397] -> w53
    stop <- w398 stop-if-true
    # "Fetch buffer data and parse dataframes"
    n141 = Wait (ms)(milliseconds to wait=u32 100) -> ()  [unwired: 1 out]
    n142 = VISA Write(VISA resource name=w396, write buffer="*OPC", error in (no error)=w395) -> (VISA resource name out=w408:refnum<visa-resource-name>, error out=w407:errorcluster)  [unwired: 1 out]
    n143 = call <instrlib>:"ESR.vi"("error in (no error)"=w407, "VISA resource name"=w408) -> ("error out"=w402:errorcluster, "ESR"=w406:u8, "VISA resource name out"=w401:refnum<visa-resource-name>)  [unwired: 5 in, 2 out]
    n144 = And(x=w406, y=u8 1) -> (x .and. y?=w405:u8)
    n145 = Not Equal To 0?(x=w405) -> (x != 0?=w397:bool)
    "Complete?" <- w397
    n146 = call <instrlib>:"Print.vi"("Byte Count (1024)"=u32 256, "error in (no error)"=w402, "Input"=w410, "VISA resource name"=w401) -> ("error out"=w419:errorcluster, "Output"=w421:string, "VISA resource name out"=w416:refnum<visa-resource-name>)  [unwired: 3 in, 2 out]
    n147 = Scan From String(format string="%d %d", input string=w421, error in=w419) -> (error out=w415:errorcluster, output 1=w418:i32, output 2=w417:i32)  [unwired: 3 in, 2 out]
    n148 = Max & Min(x=w418, y=w417) -> (min(x,y)=w390:i32)  [unwired: 1 out]
    n149 = Decrement(x=w390) -> (x-1=w400:i32)
    n150 = Greater Or Equal?(x=w390, y=w389) -> (x >= y?=w414:bool)
    n151 = Equal?(x=w390, y=w389) -> (x = y?=w388:bool)
    n152 = case shown="False" w414 {
      tunnel: w412 -> [w428 w455]
      tunnel: w416 -> [w431 w454]
      tunnel: w415 -> [w432 w453]
      tunnel: w400 -> [w438 w452]
      tunnel: w389 -> [w445 w451]
      tunnel: u32 4096 ("Byte Count (1024)") -> [w444 w450]
      tunnel: [w434 w449] -> w392
      tunnel: [w427 w447] -> w393
      tunnel: [w426 w448] -> w409
      tunnel: w388 -> [_ w446]
      frame False {
        n153 = VISA Write(VISA resource name=w431, write buffer="i_ds.clearcache()\nv_ds.clearcache()" ("format string"), error in (no error)=w432) -> (VISA resource name out=w430:refnum<visa-resource-name>, error out=w429:errorcluster)  [unwired: 1 out]
        n154 = local read "Buffer size"() -> (w443:u32)
        n155 = call <instrlib>:"Print Buffer.vi"("VISA resource name"=w430, "Start Index (1)"=w445, "End Index (1)"=w443, "Buffer Name(s)"=w428, "error in (no error)"=w429, "Byte Count (1024)"=w444) -> ("VISA resource name out"=w441:refnum<visa-resource-name>, "Buffer Data"=w442:string, "error out"=w440:errorcluster)  [unwired: 5 in, 2 out]
        n156 = call <instrlib>:"Real 32 Converter.vi"("Data In"=w442) -> ("Data Array Out"=w436:sgl[])  [unwired: 10 in]
        n157 = call <instrlib>:"Print Buffer.vi"("VISA resource name"=w441, "Start Index (1)"=u32 1, "End Index (1)"=w438, "Buffer Name(s)"=w428, "error in (no error)"=w440) -> ("VISA resource name out"=w426:refnum<visa-resource-name>, "Buffer Data"=w437:string, "error out"=w427:errorcluster)  [unwired: 6 in, 2 out]
        n158 = call <instrlib>:"Real 32 Converter.vi"("Data In"=w437) -> ("Data Array Out"=w435:sgl[])  [unwired: 10 in]
        n159 = Build Array (concatenate)(w436, w435) -> (w434:sgl[])
      }
      frame True {
        n160 = case shown="True" w446 {
          tunnel: w455 -> [w465 _]
          tunnel: w454 -> [w464 w468]
          tunnel: w453 -> [w463 w467]
          tunnel: w452 -> [w462 _]
          tunnel: w451 -> [w461 _]
          tunnel: w450 -> [w460 _]
          tunnel: [w458 sgl[] [] ("Data Array Out")] -> w449
          tunnel: [w457 w468] -> w448
          tunnel: [w456 w467] -> w447
          frame False {
            n161 = call <instrlib>:"Print Buffer.vi"("VISA resource name"=w464, "Start Index (1)"=w461, "End Index (1)"=w462, "Buffer Name(s)"=w465, "error in (no error)"=w463, "Byte Count (1024)"=w460) -> ("VISA resource name out"=w457:refnum<visa-resource-name>, "Buffer Data"=w459:string, "error out"=w456:errorcluster)  [unwired: 5 in, 2 out]
            n162 = call <instrlib>:"Real 32 Converter.vi"("Data In"=w459) -> ("Data Array Out"=w458:sgl[])  [unwired: 10 in]
          }
          frame True {
          }
        }
      }
    }
    n163 = Empty Array?(array=w392) -> (empty?=w391:bool)
    n164 = case shown="False" w391 {
      tunnel: w394 -> [w424 _]
      tunnel: w392 -> [w423 _]
      frame False {
        n165 = Lossy Enqueue Element(queue=w424, element=w423) -> (overflow?=→"Overflow?":bool)  [unwired: 1 in, 3 out]
      }
      frame True {
      }
    }
    n166 = Or(x=w397, y="Stop") -> (x .or. y?=w398:bool)
  }
  n167 = Release Queue(queue=w29) -> (error out=w26:errorcluster)  [unwired: 2 in, 2 out]
  n168 = Decimate 1D Array(w15) -> (w18:sgl[], w17:sgl[], w16:sgl[])
  n169 = for {
    tunnel: w18 -> [w474] mode=indexing
    tunnel: w17 -> [w470] mode=indexing
    tunnel: w16 -> [w473] mode=indexing
    n170 = To Time Stamp(1:w470) -> (0:w475:timestamp)
    n171 = Build Array(w474) -> (w472:sgl[])
    n172 = Build Array(w473) -> (w471:sgl[])
    n173 = Bundle By Name("Y"=w472, "t0"=w475) -> (w477:waveform(sgl))  [unwired: 1 in]
    n174 = Bundle By Name("Y"=w471, "t0"=w475) -> (w476:waveform(sgl))  [unwired: 1 in]
    n175 = Merge Signals(w477, w476) -> (w469:dynamicdata)
    n176 = local write "Result Chart"(w469) -> ()
  }
  n177 = case shown="False" w53 {
    tunnel: w61 -> [w485 w487]
    tunnel: w60 -> [w484 w486]
    tunnel: [w479 w487] -> w59
    tunnel: [w478 w486] -> w58
    frame False {
      w480 = u16 1 items=["Channel A", "Channel B"] ("Channel (Channel A)")
      w481 = u16 0 items=["Channel A", "Channel B"] ("Channel (Channel A)")
      # "Abort Operation"
      n178 = call <instrlib>:"Abort SMU Op.vi"("error in"=w484, "Channel (Channel A)"=w481, "VISA resource name"=w485) -> ("error out"=w482:errorcluster, "VISA resource name out"=w483:refnum<visa-resource-name>)  [unwired: 5 in, 2 out]
      n179 = call <instrlib>:"Abort SMU Op.vi"("error in"=w482, "Channel (Channel A)"=w480, "VISA resource name"=w483) -> ("error out"=w478:errorcluster, "VISA resource name out"=w479:refnum<visa-resource-name>)  [unwired: 5 in, 2 out]
    }
    frame True {
      # "Operation Completed"
    }
  }
  n180 = local read "Auto Enable Output"() -> (w11:bool)
  n181 = case shown="False" w11 {
    tunnel: w59 -> [w489 w493]
    tunnel: w58 -> [w488 w492]
    tunnel: [w488 w491] -> w55
    tunnel: [w489 w490] -> w54
    frame False {
    }
    frame True {
      w498 = FALSE ("Output (Off)")
      n182 = local read "Drain Source Channel"() -> (w495:T1)
      n183 = local read "Pulse Channel"() -> (w494:T1)
      n184 = call <instrlib>:"Source Output Enable.vi"("Output (Off)"=w498, "error in (no error)"=w492, "Channel (Channel A)"=w495, "VISA resource name"=w493) -> ("error out"=w496:errorcluster, "VISA resource name out"=w497:refnum<visa-resource-name>)  [unwired: 4 in, 2 out]
      n185 = call <instrlib>:"Source Output Enable.vi"("Output (Off)"=w498, "error in (no error)"=w496, "Channel (Channel A)"=w494, "VISA resource name"=w497) -> ("error out"=w491:errorcluster, "VISA resource name out"=w490:refnum<visa-resource-name>)  [unwired: 4 in, 2 out]
    }
  }
  n186 = case shown="True" w53 {
    tunnel: w55 -> [w499 w518]
    tunnel: w54 -> [w500 w517]
    tunnel: [w499 w506] -> w52
    tunnel: [w500 w512] -> w51
    frame False {
      # "Operation Aborted, do nothing"
    }
    frame True {
      # "Plot and save Pulsed IV (single point)"
      n187 = local read "Pulse Number"() -> (w514:u32)
      n188 = call <instrlib>:"Print Buffer.vi"("VISA resource name"=w517, "End Index (1)"=w514, "Buffer Name(s)"="pulse_iv_table.v, pulse_iv_table.i" ("Buffer Name (buf)"), "error in (no error)"=w518, "Byte Count (1024)"=u32 4096) -> ("VISA resource name out"=w512:refnum<visa-resource-name>, "Buffer Data"=w513:string, "error out"=w507:errorcluster)  [unwired: 6 in, 2 out]
      n189 = call <instrlib>:"Real 32 Converter.vi"("Data In"=w513) -> ("Data Array Out"=w511:sgl[])  [unwired: 10 in]
      n190 = Decimate 1D Array(w511) -> (w510:sgl[], w509:sgl[])
      n191 = call "Convert to Dynamic Data2"("Array"=w509) -> ("Dynamic Data Type"=w504:dynamicdata)  [unwired: 3 in]
      n192 = call "Convert to Dynamic Data"("Array"=w510) -> ("Dynamic Data Type"=w505:dynamicdata)  [unwired: 3 in]
      n193 = Merge Signals(w505, w504) -> (w501:dynamicdata)
      n194 = call "Build XY Graph"("error in (no error)"=w507, "Y Input"=w504, "X Input"=w505) -> ("error out"=w506:errorcluster, "XY Graph"=→"Pulse IV":cluster{"X":dbl[], "Y":dbl[]}[])  [unwired: 7 in]
      n195 = call "Write To Measurement File2"("Signals"=w501, "Filename"="Pulsed IV Filename") -> ("Filename Out"=→"Pulsed IV Filename Out":path)  [unwired: 15 in, 2 out]
    }
  }
  n196 = call <instrlib>:"Close.vi"("error in (no error)"=w52, "VISA resource name"=w51) -> ("error out"=w28:errorcluster)  [unwired: 9 in]
  n197 = Merge Errors(w28, w26) -> (→"error out":errorcluster)
